vi "Update Filter Arguments.vi"(8 "error in (no error)":errorcluster caption="错误输入（无错误）", 11 "Data Viewer 输入":refnum<class "Data Viewer.lvclass">) -> (0 "error out":errorcluster caption="错误输出", 3 "Data Viewer 输出":refnum<class "Data Viewer.lvclass">)   [LabVIEW 2020, in "Data Viewer.lvlib" / "Data Viewer.lvclass"]
uses:
  Data Viewer.lvclass
  Data Viewer.lvclass/Data Viewer.ctl
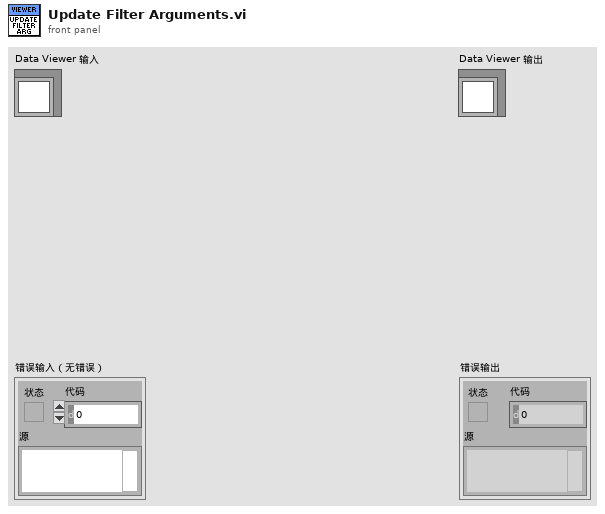
[diagram p1: front panel]
types:
  T1 = typedef "DataSave.lvlib/Data Viewer.lvlib/Data Viewer.lvclass/Filter Type.ctl" = enum16{"Butterworth滤波器", "中值滤波器"}
  T2 = typedef "Filte Method.ctl" = enum16{"低通", "高通", "带通", "带阻"}
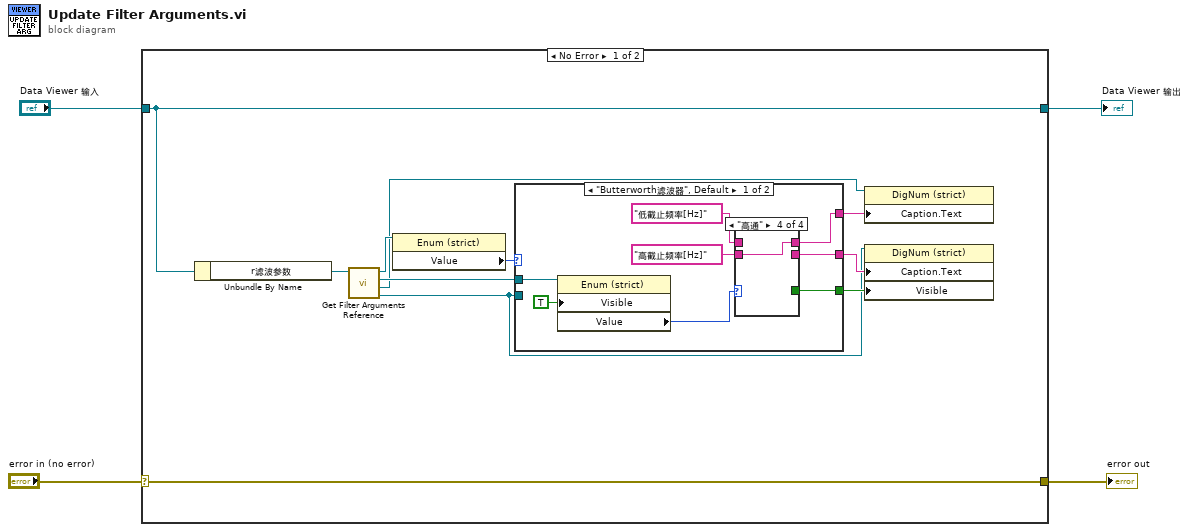
[diagram p0: block diagram]
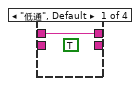
[diagram p2: hidden frame]
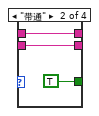
[diagram p3: hidden frame]
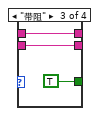
[diagram p4: hidden frame]
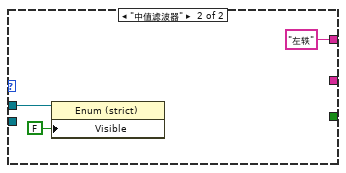
[diagram p5: hidden frame]
diagram:
  n1 = case shown="No Error" "error in (no error)" {
    selector: "error in (no error)" -> [w15 w36]
    tunnel: [w15 w36] -> w3
    tunnel: [w14 w35] -> w1
    tunnel: "Data Viewer 输入" -> [w14 w35]
    frame No Error {
      n2 = Unbundle By Name(w14) -> ("r滤波参数"=w13:refnum<vi>)
      n3 = call "Get Filter Arguments Reference.vi"("滤波参数引用"=w13) -> ("参数2"=w5:refnum<vi>, "参数1"=w6:refnum<vi>, "滤波方式"=w7:refnum<vi>, "滤波器类型"=w9:refnum<vi>)  [unwired: 7 in]
      n4 = property class="Enum (strict)"(reference=w9) -> ("Value"=w8:T1)  [unwired: 1 in, 2 out]
      n5 = case shown="\"Butterworth滤波器\", Default" w8 {
        tunnel: w7 -> [w23 w33]
        tunnel: w5 -> [_ _]
        tunnel: [w18 _] -> w12
        tunnel: [w17 _] -> w11
        tunnel: [w16 "左轶"] -> w10
        frame "Butterworth滤波器", Default {
          n6 = property class="Enum (strict)"(reference=w23, "Visible"=TRUE) -> ("Value"=w21:T2)  [unwired: 1 in, 2 out]
          n7 = case shown="\"高通\"" w21 {
            tunnel: [w24 w27 w30 w31] -> w16
            tunnel: "低截止频率[Hz]" -> [w24 w27 w30 _]
            tunnel: "高截止频率[Hz]" -> [_ w26 w29 w31]
            tunnel: [_ TRUE TRUE _] -> w17
            tunnel: [_ w26 w29 _] -> w18
            frame "低通", Default {
              (unwired) TRUE
            }
            frame "带通" {
            }
            frame "带阻" {
            }
            frame "高通" {
            }
          }
        }
        frame "中值滤波器" {
          n8 = property class="Enum (strict)"(reference=w33, "Visible"=FALSE ("可见")) -> ()  [unwired: 1 in, 2 out]
        }
      }
      n9 = property class="DigNum (strict)"(reference=w6, "Caption.Text"=w10) -> ()  [unwired: 1 in, 2 out]
      n10 = property class="DigNum (strict)"(reference=w5, "Caption.Text"=w12, "Visible"=w11) -> ()  [unwired: 1 in, 2 out]
    }
    frame Error {
    }
  }
  "error out" <- w3
  "Data Viewer 输出" <- w1
